vi "Parameter XML Write (Ballard-1533).vi"(6 "ballard_bus hw map":T1, 8 "error in":errorcluster caption="error out", 10 "configuration":T3[](array[typedef]), 11 "parameter file in":refnum<k24>) -> (0 "error out":errorcluster, 3 "parameter file out":refnum<k24>)   [LabVIEW 2020]
uses:
  _controls/ballard1553_cluster.ctl
  _controls/aim1553_messages.ctl
  _controls/1553_Parameters_key.ctl
  _controls/1553_Parameters.ctl
  _controls/1553_minorFrames.ctl
  C:/Users/Administrator/Desktop/GIT/Ballard-Arinc-429-XML-Generator/Source/Assemblies/Ballard_1553_Parameter_ni/bin/Debug/Ballard_1553_Parameter_ni.dll
  Assemblies/Ballard_1553_Parameter_ni/bin/Debug/Ballard_1553_Parameter_ni.dll
  _controls/ballard1553_hw_map.ctl
  _controls/ballard1553_RT_list.ctl
  Libraries/Ballard_1553_Parameter_ni/_tyedefs/message_type.ctl
  Libraries/Ballard_1553_Parameter_ni/_tyedefs/messageAddress_type.ctl
  Libraries/Ballard_1553_Parameter_ni/_tyedefs/parameter_type.ctl
  Libraries/Ballard_1553_Parameter_ni/Ballard_1553_Parameter_ni.lvlib
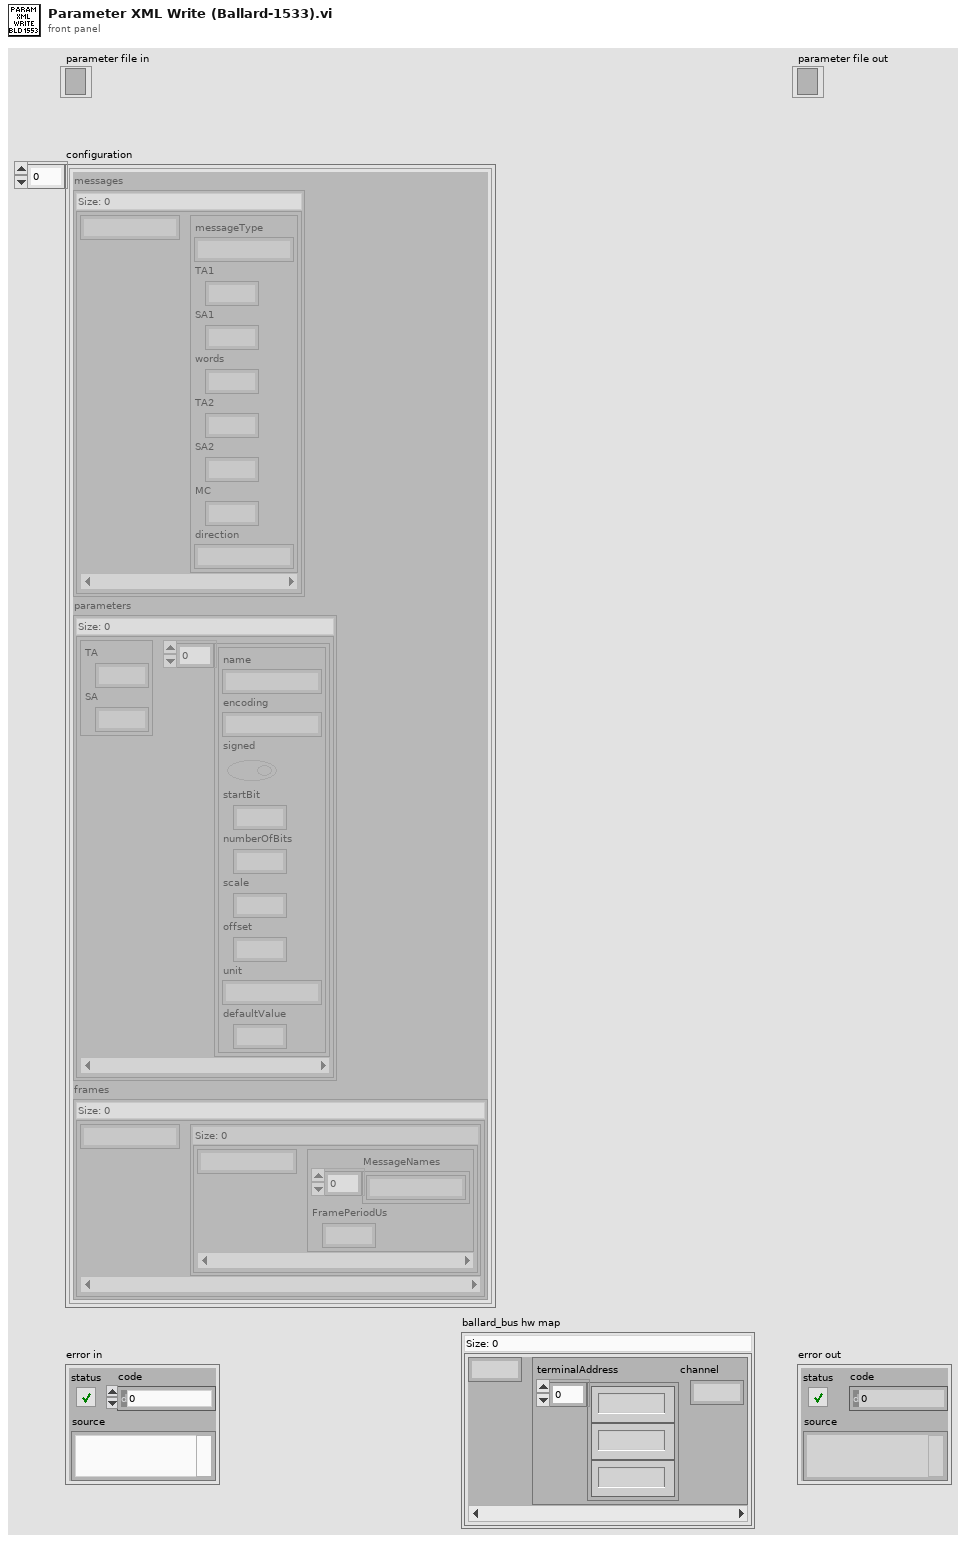
[diagram p1: front panel]
types:
  T1 = typedef "ballard1553_hw_map.ctl" = map{i32, T2}
  T2 = typedef "ballard1553_RT_list.ctl" = cluster{"terminalAddress":i32[], "channel":i32}
  T3 = typedef "ballard1553_cluster.ctl" = cluster{"messages":map{string, T4}, "parameters":map{T5, T6[]}, "frames":map{string, map{string, T7}}}
  T4 = typedef "aim1553_messages.ctl" = cluster{"messageType":string, "TA1":i32, "SA1":i32, "words":i32, "TA2":i32, "SA2":i32, "MC":i32, "direction":string}
  T5 = typedef "1553_Parameters_key.ctl" = cluster{"TA":i32, "SA":i32}
  T6 = typedef "1553_Parameters.ctl" = cluster{"name":string, "encoding":string, "signed":bool, "startBit":i32, "numberOfBits":i32, "scale":dbl, "offset":dbl, "unit":string, "defaultValue":dbl}
  T7 = typedef "1553_minorFrames.ctl" = cluster{"MessageNames":string[], "FramePeriodUs":i32}
  T8 = typedef "Ballard_1553_Parameter_ni.lvlib/message_type.ctl" = cluster{"name":string, "numberOfWords":i32, "modeCode":i32, "messageType":i32, "createTimestampChannel":bool, "modeCodeSpecified":bool}
  T9 = typedef "Ballard_1553_Parameter_ni.lvlib/parameter_type.ctl" = cluster{"defaultValue":dbl, "encoding":i32, "name":string, "numberOfBits":i32, "offset":dbl, "scale":dbl, "signed":bool, "startBit":i32, "unit":string}
  T10 = typedef "Ballard_1553_Parameter_ni.lvlib/messageAddress_type.ctl" = cluster{"direction":i32, "subAddress":i32, "terminalAddress":i32}
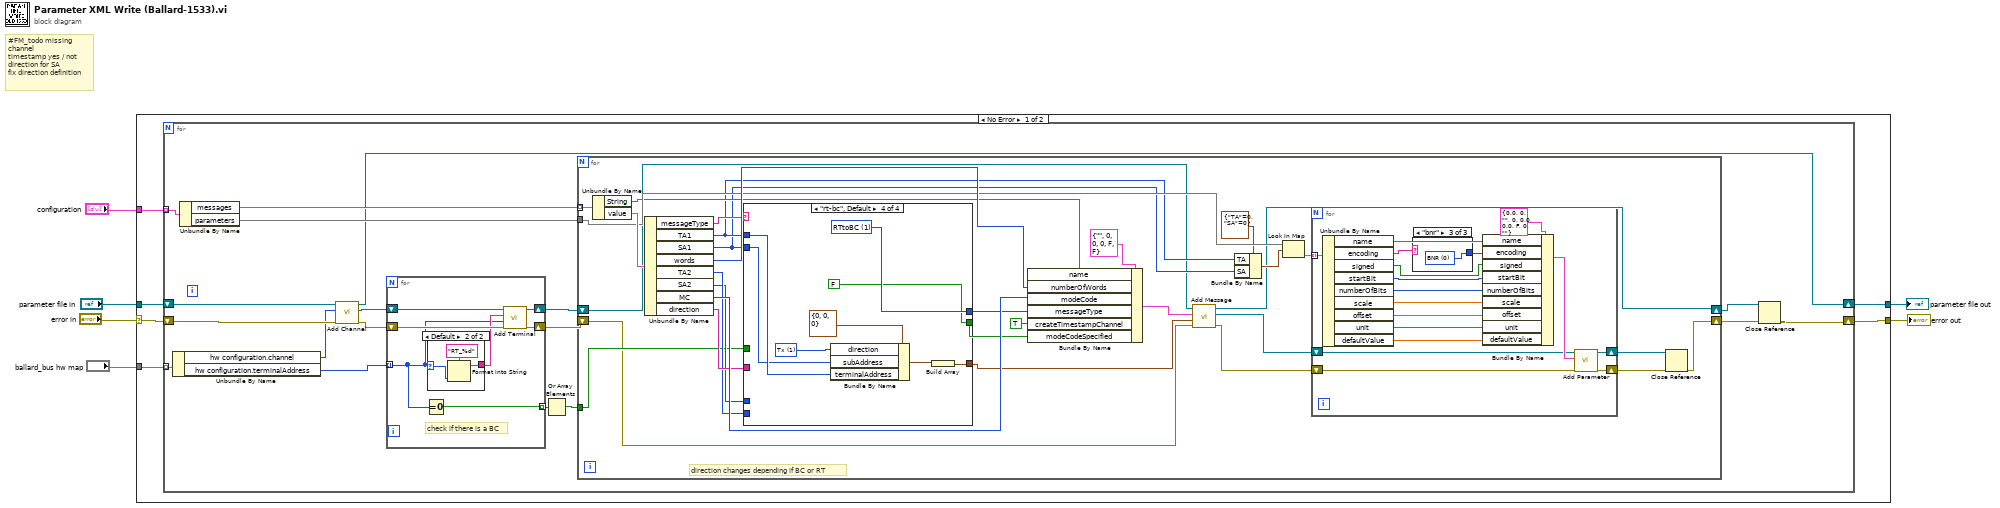
[diagram p0: block diagram]
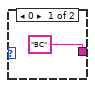
[diagram p2: hidden frame]
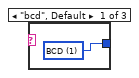
[diagram p3: hidden frame]
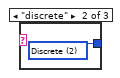
[diagram p4: hidden frame]
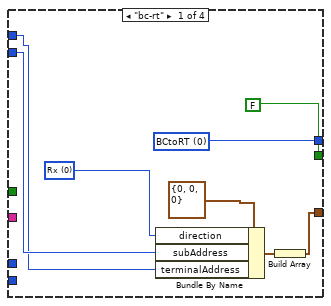
[diagram p5: hidden frame]
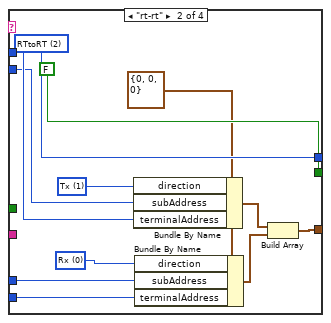
[diagram p6: hidden frame]
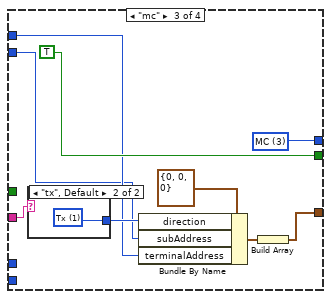
[diagram p7: hidden frame]
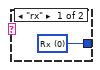
[diagram p8: hidden frame]
diagram:
  # "#FM_todo missing \nchannel\ntimestamp yes / not\ndirection for SA\nfix direction definition"
  n1 = case shown="No Error" "error in" {
    selector: "error in" -> [w11 w132]
    tunnel: "configuration" -> [w10 _]
    tunnel: "parameter file in" -> [w12 w131]
    tunnel: [w8 w132] -> w3
    tunnel: [w9 w131] -> w2
    tunnel: "ballard_bus hw map" -> [w7 _]
    frame No Error {
      n2 = for {
        tunnel: w10 -> [w29] mode=indexing
        tunnel: w7 -> [w25] mode=indexing
        shift-right: [w14] -> w9
        shift-left: w12 -> [w21]
        shift-right: [w15] -> w8
        shift-left: w11 -> [w20]
        n3 = Unbundle By Name(w25) -> ("hw configuration.channel"=w13:i32, "hw configuration.terminalAddress"=w24:i32[])
        n4 = Unbundle By Name(w29) -> ("messages"=w30:map{string, T4}, "parameters"=w28:map{T5, T6[]})
        n5 = call "Add Channel.vi"("error in"=w20, "hardwareChannel"=w13, "parameter file in"=w21) -> ("error out"=w19:errorcluster, "new channel"=w18:refnum<k24>, "parameter file out"=w14:refnum<k24>)  [unwired: 6 in]
        n6 = for {
          shift-right: [w32] -> w27
          shift-left: w19 -> [w35]
          shift-right: [w31] -> w26
          shift-left: w18 -> [w36]
          tunnel: w24 -> [w33] mode=indexing
          tunnel: [w37] -> w23 mode=indexing
          # "check if there is a BC"
          n7 = Equal To 0?(x=w33) -> (x = 0?=w37:bool)
          n8 = case shown="Default" w33 {
            selector: w33 -> [_ w40]
            tunnel: ["BC" ("BC") w41] -> w34
            frame 0 {
            }
            frame Default {
              n9 = Format Into String(format string="RT_%d", w40) -> (resulting string=w41:string)  [unwired: 2 in, 1 out]
            }
          }
          n10 = call "Add Terminal.vi"("error in"=w35, "terminalAddress"=w33, "name"=w34, "channel in"=w36) -> ("error out"=w32:errorcluster, "channel out"=w31:refnum<k24>)  [unwired: 5 in, 1 out]
        }
        n11 = Or Array Elements(Boolean array=w23) -> (logical OR=w22:bool)
        n12 = for {
          tunnel: w30 -> [w71] mode=indexing
          tunnel: w28 -> [w58]
          shift-right: [w43] -> w17
          shift-left: w26 -> [w44]
          shift-right: [w51] -> w16
          shift-left: w27 -> [w49]
          tunnel: w22 -> [w50]
          # "direction changes depending if BC or RT"
          n13 = Unbundle By Name(w71) -> ("String"=w57:string, "value"=w70:T4)
          n14 = Unbundle By Name(w70) -> ("messageType"=w68:string, "TA1"=w54:i32, "SA1"=w53:i32, "words"=w69:i32, "TA2"=w60:i32, "SA2"=w59:i32, "MC"=w67:i32, "direction"=w63:string)
          n15 = case shown="\"rt-bc\", Default" w68 {
            tunnel: [w99 w111 w120 w130] -> w65
            tunnel: [FALSE FALSE TRUE FALSE] -> w64
            tunnel: w63 -> [_ _ w117 _]
            tunnel: w54 -> [w96 w104 w115 w127]
            tunnel: w53 -> [w97 w103 w114 w126]
            tunnel: [w94 w106 w113 w124] -> w42
            tunnel: w60 -> [_ w102 _ _]
            tunnel: w59 -> [_ w101 _ _]
            tunnel: w50 -> [_ _ _ _]
            frame "bc-rt" {
              w93 = 0 items=["Rx", "Tx"] ("direction")
              w99 = 0 items=["BCtoRT", "RTtoBC", "RTtoRT", "MC"] ("messageType")
              n16 = Bundle By Name(cluster=T10 {"direction"=0, "subAddress"=0, "terminalAddress"=0} ("messageAddress"), "direction"=w93, "subAddress"=w97, "terminalAddress"=w96) -> (w95:T10)
              n17 = Build Array(w95) -> (w94:T10[])
            }
            frame "rt-rt" {
              w100 = T10 {"direction"=0, "subAddress"=0, "terminalAddress"=0} ("messageAddress")
              w105 = 0 items=["Rx", "Tx"] ("direction")
              w109 = 1 items=["Rx", "Tx"] ("direction")
              w111 = 2 items=["BCtoRT", "RTtoBC", "RTtoRT", "MC"] ("messageType")
              n18 = Bundle By Name(cluster=w100, "direction"=w109, "subAddress"=w103, "terminalAddress"=w104) -> (w108:T10)
              n19 = Bundle By Name(cluster=w100, "direction"=w105, "subAddress"=w101, "terminalAddress"=w102) -> (w107:T10)
              n20 = Build Array(w108, w107) -> (w106:T10[])
            }
            frame "mc" {
              w120 = 3 items=["BCtoRT", "RTtoBC", "RTtoRT", "MC"] ("messageType")
              n21 = case shown="\"tx\", Default" w117 {
                tunnel: [w121 w122] -> w116
                frame "rx" {
                  w121 = 0 items=["Rx", "Tx"] ("direction")
                }
                frame "tx", Default {
                  w122 = 1 items=["Rx", "Tx"] ("direction")
                }
              }
              n22 = Bundle By Name(cluster=T10 {"direction"=0, "subAddress"=0, "terminalAddress"=0} ("messageAddress"), "direction"=w116, "subAddress"=w114, "terminalAddress"=w115) -> (w118:T10)
              n23 = Build Array(w118) -> (w113:T10[])
            }
            frame "rt-bc", Default {
              w128 = 1 items=["Rx", "Tx"] ("direction")
              w130 = 1 items=["BCtoRT", "RTtoBC", "RTtoRT", "MC"] ("messageType")
              n24 = Bundle By Name(cluster=T10 {"direction"=0, "subAddress"=0, "terminalAddress"=0} ("messageAddress"), "direction"=w128, "subAddress"=w126, "terminalAddress"=w127) -> (w125:T10)
              n25 = Build Array(w125) -> (w124:T10[])
            }
          }
          n26 = Bundle By Name(cluster=T8 {"name"="", "numberOfWords"=0, "modeCode"=0, "messageType"=0, "createTimestampChannel"=FALSE, "modeCodeSpecified"=FALSE} ("message configuration"), "name"=w57, "numberOfWords"=w69, "modeCode"=w67, "messageType"=w65, "createTimestampChannel"=TRUE, "modeCodeSpecified"=w64) -> (w45:T8)
          n27 = call "Add Message.vi"("error in"=w49, "messageAddresses"=w42, "message configuration"=w45, "channel in"=w44) -> ("error out"=w48:errorcluster, "new message"=w47:refnum<k24>, "channel out"=w43:refnum<k24>)  [unwired: 5 in]
          n28 = Bundle By Name(cluster=T5 {"TA"=0, "SA"=0} ("key"), "TA"=w54, "SA"=w53) -> (w55:T5)
          n29 = Look In Map(map=w58, key=w55) -> (value=w52:T6[])  [unwired: 1 in, 1 out]
          n30 = for {
            shift-right: [w77] -> w61
            shift-left: w48 -> [w76]
            shift-right: [w72] -> w62
            shift-left: w47 -> [w73]
            tunnel: w52 -> [w88] mode=indexing
            n31 = Unbundle By Name(w88) -> ("name"=w87:string, "encoding"=w86:string, "signed"=w84:bool, "startBit"=w83:i32, "numberOfBits"=w82:i32, "scale"=w81:dbl, "offset"=w80:dbl, "unit"=w79:string, "defaultValue"=w78:dbl)
            n32 = case shown="\"bnr\"" w86 {
              tunnel: [w89 w90 w91] -> w85
              frame "bcd", Default {
                w89 = 1 items=["BNR", "BCD", "Discrete"] ("encoding")
              }
              frame "discrete" {
                w90 = 2 items=["BNR", "BCD", "Discrete"] ("encoding")
              }
              frame "bnr" {
                w91 = 0 items=["BNR", "BCD", "Discrete"] ("encoding")
              }
            }
            n33 = Bundle By Name(cluster=T9 {"defaultValue"=0.0, "encoding"=0, "name"="", "numberOfBits"=0, "offset"=0.0, "scale"=0.0, "signed"=FALSE, "startBit"=0, "unit"=""} ("parameter configuration"), "name"=w87, "encoding"=w85, "signed"=w84, "startBit"=w83, "numberOfBits"=w82, "scale"=w81, "offset"=w80, "unit"=w79, "defaultValue"=w78) -> (w74:T9)
            n34 = call "Add Parameter.vi"("error in"=w76, "parameter configuration"=w74, "message in"=w73) -> ("error out"=w77:errorcluster, "message out"=w72:refnum<k24>)  [unwired: 6 in, 1 out]
          }
          n35 = Close Reference(reference=w62, error in (no error)=w61) -> (error out=w51:errorcluster)
        }
        n36 = Close Reference(reference=w17, error in (no error)=w16) -> (error out=w15:errorcluster)
      }
    }
    frame Error {
    }
  }
  "error out" <- w3
  "parameter file out" <- w2
